vi "2_Analog_Meter_Reader(Evaluation).vi"() -> ()   [LabVIEW 2020]
uses:
  Controls/Regression_Report.ctl
  <vilib>/Ngene/Deep Learning Toolkit/Toolkit/NN_Network/Controls/NN_Save_Before_Destroy_Options.ctl
  <vilib>/Ngene/Deep Learning Toolkit/Toolkit/NN_Network/subVIs/NN_Predict/NN_Predict(In3D_Out1D).vi
  <vilib>/Ngene/Deep Learning Toolkit/Toolkit/Deep_Learning_Toolkit_by_Ngene.lvlib
panel:
  in  "Image Folder(Test)":path=path "D:/working/Analog_Meter/Test/Images"
  in  "Labels (Test)":path=path "D:/working/Analog_Meter/Test/Labels.csv"
  in  "NN Device":enum16{"CPU", "GPU"}(ring)=enum."GPU"
  in  "Image Folder(Train)":path=path "D:/working/Analog_Meter/Train/Images"
  in  "Labels (Train)":path=path "D:/working/Analog_Meter/Train/Labels.csv"
  out "Metrics (Test)":T1={"Graphs"=[{"Best Linear Fit"=[0.0, 0.7035179734230042, 1.407034993171692, 2.110553026199341, 2.814069986343384, 3.517587900161743, 4.221106052398682, 4.924623012542725, 5.628140926361084, 6.331657886505127, 7.035175800323486, 7.7386932373046875, 8.442211151123047, 9.145729064941406, 9.84924602508545, 10.552763938903809, 11.256280899047852, 11.959798812866211, 12.66331672668457, 13.366833686828613, 14.070351600646973, 14.773868560791016, 15.477387428283691, 16.180904388427734, 16.884422302246094, 17.587940216064453, 18.29145622253418, 18.99497413635254, 19.6984920501709, 20.402009963989258, 21.105527877807617, 21.809045791625977, 22.512563705444336, 23.216079711914062, 23.919597625732422, 24.62311553955078, 25.32663345336914, 26.0301513671875, 26.733667373657227, 27.437185287475586, 28.140703201293945, 28.844221115112305, 29.547739028930664, 30.251256942749023, 30.954774856567383, 31.65829086303711, 32.36180877685547, 33.06532669067383, 33.76884460449219, 34.47236251831055, 35.175880432128906, 35.879398345947266, 36.582916259765625, 37.28643035888672, 37.98994827270508, 38.69346618652344, 39.3969841003418, 40.100502014160156, 40.804019927978516, 41.507537841796875, 42.211055755615234, 42.914573669433594, 43.61809158325195, 44.32160949707031, 45.02512741088867, 45.728641510009766, 46.432159423828125, 47.135677337646484, 47.839195251464844, 48.5427131652832, 49.24623107910156, 49.94974899291992, 50.65326690673828, 51.35678482055664, 52.060302734375, 52.76382064819336, 53.46733856201172, 54.17085266113281, 54.87437057495117, 55.57788848876953, 56.28140640258789, 56.98492431640625, 57.68844223022461, 58.39196014404297, 59.09547805786133, 59.79899597167969, 60.50251388549805, 61.206031799316406, 61.909549713134766, 62.61306381225586, 63.31658172607422, 64.02010345458984, 64.72361755371094, 65.42713928222656, 66.13065338134766, 66.83416748046875, 67.53768920898438, 68.24120330810547, 68.9447250366211, 69.64823913574219, 70.35176086425781, 71.0552749633789, 71.75879669189453, 72.46231079101562, 73.16583251953125, 73.86934661865234, 74.57286071777344, 75.27638244628906, 75.97989654541016, 76.68341827392578, 77.38693237304688, 78.0904541015625, 78.7939682006836, 79.49748992919922, 80.20100402832031, 80.90452575683594, 81.60803985595703, 82.31156158447266, 83.01507568359375, 83.71858978271484, 84.42211151123047, 85.12562561035156, 85.82914733886719, 86.53266143798828, 87.2361831665039, 87.939697265625, 88.64321899414062, 89.34673309326172, 90.05024719238281, 90.75376892089844, 91.45728302001953, 92.16080474853516, 92.86431884765625, 93.56784057617188, 94.27135467529297, 94.9748764038086, 95.67839050292969, 96.38191223144531, 97.0854263305664, 97.78894805908203, 98.49246215820312, 99.19597625732422, 99.89949798583984, 100.60301208496094, 101.30653381347656, 102.01004791259766, 102.71356964111328, 103.41708374023438, 104.12060546875, 104.8241195678711, 105.52764129638672, 106.23115539550781, 106.9346694946289, 107.63819122314453, 108.34170532226562, 109.04522705078125, 109.74874114990234, 110.45226287841797, 111.15577697753906, 111.85929870605469, 112.56281280517578, 113.2663345336914, 113.9698486328125, 114.67337036132812, 115.37688446044922, 116.08039855957031, 116.78392028808594, 117.48743438720703, 118.19095611572266, 118.89447021484375, 119.59799194335938, 120.30150604248047, 121.0050277709961, 121.70854187011719, 122.41206359863281, 123.1155776977539, 123.819091796875, 124.52261352539062, 125.22612762451172, 125.92964935302734, 126.63316345214844, 127.33668518066406, 128.0402069091797, 128.74371337890625, 129.44723510742188, 130.1507568359375, 130.85427856445312, 131.5577850341797, 132.2613067626953, 132.96482849121094, 133.6683349609375, 134.37185668945312, 135.07537841796875, 135.77890014648438, 136.48240661621094, 137.18592834472656, 137.8894500732422, 138.5929718017578, 139.29647827148438, 140.0], "Array 3"=[2.1188226, 0.6589031, 1.929399, 2.432055, 2.4883072, 4.273648, 4.5083437, 5.706398, 5.9845705, 6.8059487, 7.432598, 7.994937, 8.78134, 9.417916, 10.277919, 10.736919, 11.286387, 11.683645, 13.034748, 13.586398, 14.125502, 15.080678, 15.584784, 16.422787, 17.089712, 17.690838, 17.784813, 18.926296, 19.709845, 20.683924, 21.649845, 22.522131, 22.717022, 22.988167, 23.577866, 24.204796, 25.393421, 25.715101, 26.404657, 27.686317, 28.289326, 28.841589, 29.523317, 30.209864, 31.038189, 31.62104, 32.218918, 32.86568, 33.492226, 33.975018, 35.333164, 36.030624, 36.599304, 37.123245, 37.91281, 38.50647, 39.085773, 39.85792, 40.96582, 41.15784, 41.639145, 42.434624, 43.35258, 44.505047, 45.25479, 46.004475, 46.779327, 47.277832, 47.861965, 48.508224, 48.970665, 49.554684, 50.45885, 51.149567, 52.214775, 52.91149, 53.535484, 54.2692, 55.005424, 55.659153, 56.401833, 56.88768, 57.88916, 58.370445, 59.22025, 59.84033, 60.424416, 61.191326, 61.82804, 62.630703, 63.13528, 64.011055, 64.73326, 65.51304, 66.41066, 67.34145, 67.8642, 68.267624, 69.247025, 69.374054, 70.29242, 71.4705, 72.27113, 72.63514, 73.22334, 74.1789, 74.79071, 75.46382, 76.0464, 76.79272, 77.32794, 77.795815, 78.34952, 79.27538, 80.03403, 80.65024, 81.92115, 82.61013, 83.241745, 83.793884, 84.675995, 85.672966, 86.3496, 86.88513, 87.43958, 88.04053, 89.190544, 90.360306, 90.99581, 91.4058, 91.692024, 91.96738, 92.47056, 93.27053, 93.939445, 94.78347, 95.663124, 96.47722, 97.483086, 97.98357, 98.58458, 98.99364, 99.654144, 100.27281, 100.90177, 102.2082, 102.532715, 102.93065, 103.456696, 103.85712, 105.56393, 106.15371, 106.93291, 107.80965, 108.29768, 109.04674, 109.87249, 110.62822, 111.24165, 111.70335, 112.376274, 113.187935, 113.69866, 114.51671, 115.66236, 116.61186, 117.31742, 117.53223, 117.78139, 118.74351, 119.38972, 120.17767, 120.90461, 121.91789, 122.35366, 123.190186, 123.76372, 124.78726, 125.52582, 125.96348, 126.331276, 127.12903, 128.17912, 128.88647, 129.19507, 129.93562, 130.9175, 130.79819, 131.62247, 133.0474, 133.42068, 134.0507, 134.65678, 135.86343, 136.04608, 137.67035, 137.70903, 138.1547, 138.02644, 138.06976]}, {"Best Linear Fit"=[1.920118723467626, 0.456393847942531, 1.7302014113306525, 2.234167616289601, 2.2905664843931697, 4.080560696728129, 4.315868365985859, 5.517045525403783, 5.795943102197606, 6.6194623359499145, 7.247745138585171, 7.811549758789713, 8.600002296688189, 9.238238248527674, 10.10048244691285, 10.560679464305368, 11.111579746966294, 11.509873043163736, 12.864497653827364, 13.417585630938483, 13.958094364960997, 14.915760479013052, 15.42118004741793, 16.261367543190772, 16.93003137985913, 17.532723990004126, 17.626944012347625, 18.771402707127898, 19.556993457662116, 20.533611622281153, 21.502050792876176, 22.3766103341453, 22.572009312489858, 22.843860945051397, 23.43509684413774, 24.063661235940646, 25.25538483983888, 25.577903399374055, 26.269256916681858, 27.55425776900406, 28.158837839308443, 28.712540627403598, 29.396045982103374, 30.084381857940546, 30.91486624039147, 31.499236909516107, 32.09867283815002, 32.74712153667766, 33.3752996397752, 33.859349984724076, 35.22103679434274, 35.92031496707152, 36.49047709619185, 37.01578383980195, 37.80740796095711, 38.40261383703523, 38.983427590357984, 39.75758840231808, 40.8683749608405, 41.06089589709805, 41.54345463219452, 42.34100694635282, 43.26135699777041, 44.416826832973946, 45.16852553041309, 45.920163033601895, 46.69703551578084, 47.196839555555485, 47.78249530393758, 48.43043914989979, 48.89408503699591, 49.47962604615859, 50.386150021636595, 51.07866622970115, 52.14665123474088, 52.84518360254346, 53.470803021048035, 54.2064305784877, 54.94457474947321, 55.60000724182262, 56.34462270478318, 56.83173658689045, 57.835827145278245, 58.318366757171475, 59.1703857787864, 59.79208111598695, 60.37769096868128, 61.14660054903278, 61.784975144095725, 62.58972925659268, 63.095622124277654, 63.973679299418635, 64.69776791602573, 65.4795780092802, 66.37953890140763, 67.31275886860301, 67.8368646750499, 68.241343371334, 69.22329690965587, 69.35065744320725, 70.2714167311741, 71.45256520368285, 72.25528843199616, 72.62024329183221, 73.20997993178486, 74.1680294660618, 74.78143298233924, 75.45629847381701, 76.04039759345571, 76.78865793895304, 77.32527796959752, 77.79437014497523, 78.3495167349147, 79.27779526639392, 80.03841685046297, 80.65623400204727, 81.93045892934602, 82.6212349259161, 83.25449597643376, 83.80807446370787, 84.69248436696384, 85.69205420010665, 86.37045365954243, 86.90737966143868, 87.463275880945, 88.06578682065926, 89.2188012365673, 90.39161199246519, 91.02877417644297, 91.43983125464024, 91.72680169168012, 92.00287190287551, 92.5073649520836, 93.3094226929243, 93.98008107969017, 94.82630577072459, 95.70825260540376, 96.52446916592034, 97.5329580610524, 98.03474326468229, 98.63732304792819, 99.04744691380755, 99.70967579258702, 100.32995601274811, 100.96055511337532, 102.2703874450994, 102.59574962495576, 102.9947208387079, 103.52213878395526, 103.92360366340938, 105.63486262818111, 106.22618266936169, 107.00741141723779, 107.88643622646251, 108.37574545230126, 109.12675188978328, 109.95465655211767, 110.71235611073226, 111.32738892392541, 111.79028518145468, 112.46496709018139, 113.27874352996507, 113.7908017183733, 114.61098060660038, 115.75961963360803, 116.71159563853723, 117.41899352335999, 117.6343590382032, 117.88416926671499, 118.84879718290509, 119.49669130853889, 120.28670143134093, 121.01553260235053, 122.03145659890073, 122.46836059859172, 123.30706604611376, 123.88209311813732, 124.90830539802846, 125.6487864244494, 126.08758744590138, 126.45634399854075, 127.25617579852478, 128.30900757732033, 129.01820304324727, 129.32760117304227, 130.07008631116233, 131.0545182166236, 130.9348987557421, 131.76132710678667, 133.18996807557502, 133.56423211074633, 134.19589446147347, 134.80355336749884, 136.01334839845504, 136.19647219264246, 137.8249735830903, 137.8637554392528, 138.31058055678258, 138.1819961382241, 138.22542875741357], "Array 3"=[2.1188226, 0.6589031, 1.929399, 2.432055, 2.4883072, 4.273648, 4.5083437, 5.706398, 5.9845705, 6.8059487, 7.432598, 7.994937, 8.78134, 9.417916, 10.277919, 10.736919, 11.286387, 11.683645, 13.034748, 13.586398, 14.125502, 15.080678, 15.584784, 16.422787, 17.089712, 17.690838, 17.784813, 18.926296, 19.709845, 20.683924, 21.649845, 22.522131, 22.717022, 22.988167, 23.577866, 24.204796, 25.393421, 25.715101, 26.404657, 27.686317, 28.289326, 28.841589, 29.523317, 30.209864, 31.038189, 31.62104, 32.218918, 32.86568, 33.492226, 33.975018, 35.333164, 36.030624, 36.599304, 37.123245, 37.91281, 38.50647, 39.085773, 39.85792, 40.96582, 41.15784, 41.639145, 42.434624, 43.35258, 44.505047, 45.25479, 46.004475, 46.779327, 47.277832, 47.861965, 48.508224, 48.970665, 49.554684, 50.45885, 51.149567, 52.214775, 52.91149, 53.535484, 54.2692, 55.005424, 55.659153, 56.401833, 56.88768, 57.88916, 58.370445, 59.22025, 59.84033, 60.424416, 61.191326, 61.82804, 62.630703, 63.13528, 64.011055, 64.73326, 65.51304, 66.41066, 67.34145, 67.8642, 68.267624, 69.247025, 69.374054, 70.29242, 71.4705, 72.27113, 72.63514, 73.22334, 74.1789, 74.79071, 75.46382, 76.0464, 76.79272, 77.32794, 77.795815, 78.34952, 79.27538, 80.03403, 80.65024, 81.92115, 82.61013, 83.241745, 83.793884, 84.675995, 85.672966, 86.3496, 86.88513, 87.43958, 88.04053, 89.190544, 90.360306, 90.99581, 91.4058, 91.692024, 91.96738, 92.47056, 93.27053, 93.939445, 94.78347, 95.663124, 96.47722, 97.483086, 97.98357, 98.58458, 98.99364, 99.654144, 100.27281, 100.90177, 102.2082, 102.532715, 102.93065, 103.456696, 103.85712, 105.56393, 106.15371, 106.93291, 107.80965, 108.29768, 109.04674, 109.87249, 110.62822, 111.24165, 111.70335, 112.376274, 113.187935, 113.69866, 114.51671, 115.66236, 116.61186, 117.31742, 117.53223, 117.78139, 118.74351, 119.38972, 120.17767, 120.90461, 121.91789, 122.35366, 123.190186, 123.76372, 124.78726, 125.52582, 125.96348, 126.331276, 127.12903, 128.17912, 128.88647, 129.19507, 129.93562, 130.9175, 130.79819, 131.62247, 133.0474, 133.42068, 134.0507, 134.65678, 135.86343, 136.04608, 137.67035, 137.70903, 138.1547, 138.02644, 138.06976]}, {"Best Linear Fit"=[0.0, 140.0], "Array 3"=[0.0, 140.0]}], "y=k*x+b"="y = 0.997*x + 0.204", "R"=0.9999598, "R^2"=0.99991965, "MAE"=0.26860958, "MSE"=0.1448541} {"R" format="%#_7g"}
  out "Metrics (Train)":T1={"Graphs"=[{"Best Linear Fit"=array[1000 elements], "Array 3"=array[1000 elements]}, {"Best Linear Fit"=array[1000 elements], "Array 3"=array[1000 elements]}, {"Best Linear Fit"=[0.0, 140.0], "Array 3"=[0.0, 140.0]}], "y=k*x+b"="y = 0.998*x + 0.138", "R"=0.99996376, "R^2"=0.9999275, "MAE"=0.2552316, "MSE"=0.12359543} {"R" format="%#_7g"}
  in  "Network Configuration File Path":path=path "D:/Ngene/GitHub/deepltk_examples/3_Image_Processing/31_Image_Regression/working/Analog_Meter/Analog_Meter_net_cfg_24_01_29__18_13_27.cfg"
  in  "Weight File Path":path=path "D:/Ngene/GitHub/deepltk_examples/3_Image_Processing/31_Image_Regression/working/Analog_Meter/Analog_Meter_weights_24_01_29__18_13_27.bin"
  # "Overview: Performs evaluation of a trained model over Training and Tests Datasets\nInstructions:\n1. Provide paths to Train and Test datasets \n2. Provide model files (.cfg and .bin).\n2. Run the VI\n3. Drag and drop image on \"Input Image\"\n4. Observe calculated metrics on both train and test datasets."
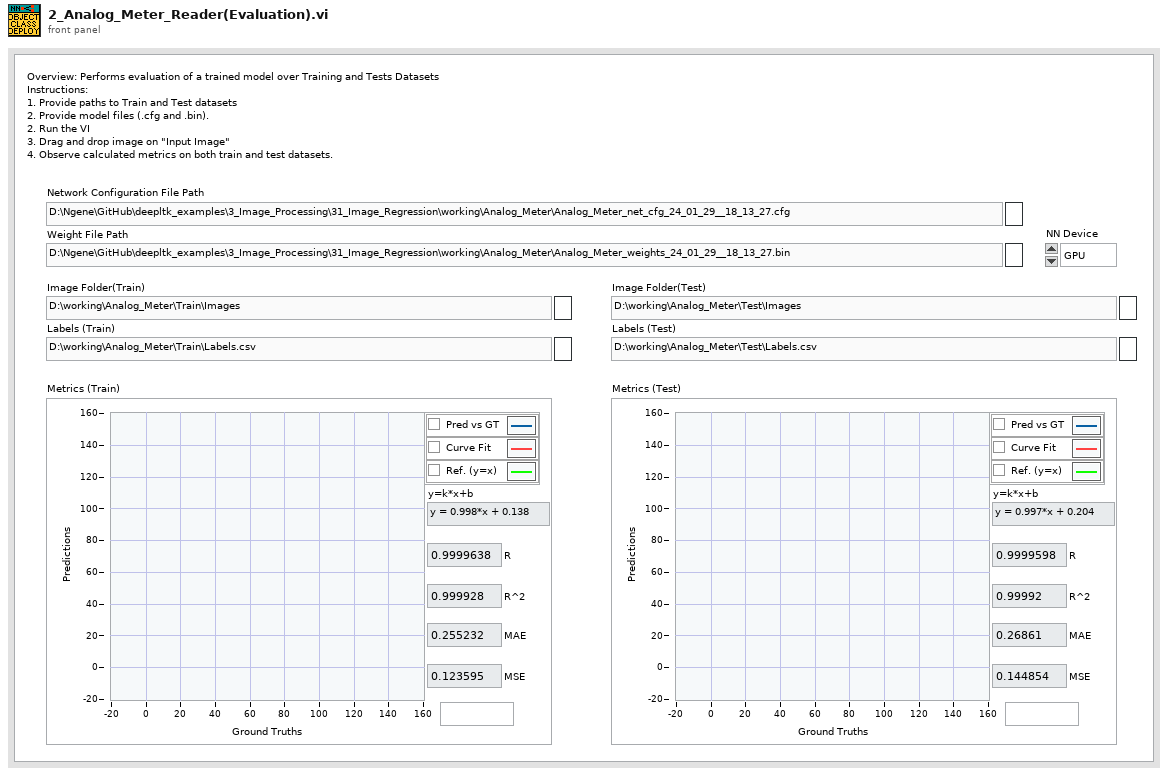
[diagram p1: front panel]
types:
  T1 = typedef "Regression_Report.ctl" = cluster{"Graphs":cluster{"Best Linear Fit":dbl[], "Array 3":sgl[]}[], "y=k*x+b":string, "R":sgl, "R^2":sgl, "MAE":sgl, "MSE":sgl}
  T2 = typedef "Deep_Learning_Toolkit_by_Ngene.lvlib/NN_Save_Before_Destroy_Options.ctl" = cluster{"CFG?":bool, "Weights?":bool, "Render?":bool}
  T3 = typedef "Deep_Learning_Toolkit_by_Ngene.lvlib/NN_Config_Params.ctl" = cluster{"Name":string, "mBatch":i32, "NN_Train_Params":T4, "LR_Decay_Policy":T7, "Labels":string[], "Loss":T9, "Max_WS_Size(B)":i64, "DryRun?":bool}
  T4 = typedef "Deep_Learning_Toolkit_by_Ngene.lvlib/NN_Train_Params.ctl" = cluster{"Optimizer":T5, "Beta_1":sgl, "Beta_2":sgl, "Weight Decay(L1)":sgl, "Weight Decay(L2)":sgl, "Data_Sampling":T6}
  T5 = typedef "Deep_Learning_Toolkit_by_Ngene.lvlib/NN_Train_Optimizer.ctl" = enum16{"SGD", "Adam", "Adagrad", "Adadelta", "RMSProp", "Nesterov"}
  T6 = typedef "Deep_Learning_Toolkit_by_Ngene.lvlib/NN_Train_Data_Sampling.ctl" = enum16{"Random", "Sequential"}
  T7 = typedef "Deep_Learning_Toolkit_by_Ngene.lvlib/NN_LR_Policy_Cfg.ctl" = cluster{"Policy_Type":T8, "LR0":dbl, "k":sgl, "WarmUp_Policy":enum16{"Step", "Ramp"}, "WarmUp_Iter":i32, "WarmUp_Ratio":sgl}
  T8 = typedef "Deep_Learning_Toolkit_by_Ngene.lvlib/NN_LR_Policy_Type.ctl" = enum16{"Manual", "Step", "Exp", "1/t"}
  T9 = typedef "Deep_Learning_Toolkit_by_Ngene.lvlib/NN_Loss_Config_Params.ctl" = cluster{"Loss_Type":T10, "Loss_Conf_Params":variant}
  T10 = typedef "Deep_Learning_Toolkit_by_Ngene.lvlib/NN_Loss_Type.ctl" = enum16{"None", "MSE", "CrossEntropy", "YOLO_v2", "YOLO_v4"}
  T11 = typedef "Deep_Learning_Toolkit_by_Ngene.lvlib/NN_Layer_Config_Params.ctl" = cluster{"Layer_Type":T12, "Layer_Conf_Params":variant, "Input Layers":string[]}
  T12 = typedef "Deep_Learning_Toolkit_by_Ngene.lvlib/NN_Layer_Type.ctl" = enum16{"Input1D", "Input3D", "Conv1D", "Conv2D", "Conv2D_Adv", "MaxPool", "AvgPool", "UpSample", "DropOut3D", "ShortCut", "Concat", "SoftMax3D", "FC", "DropOut", "Softmax", "Flatten", "YOLO_v2", "YOLO_v4", "Activation", "BatchNormalization", "LayerNormalization", "Scale", "Unsupported"}
  T13 = typedef "Deep_Learning_Toolkit_by_Ngene.lvlib/NN.ctl" = cluster{"Name":string, "No of Layers":i32, "mBatch":i32, "Layers":T14[], "Dimty":T15, "Dims_In":T16, "Dims_Out":T16, "Working_Dir":path, "Train?":bool, "Train_Params":T4, "LR_Update_Policy":T7, "Session Data":T17, "Ground_truth":T18, "NNg_hdls":T19, "NN_Device":T20, "GPU Id":i32, "Labels":string[], "Loss_Type":T10, "Loss_Cfg_Prms":variant, "NNG_WS":T21, "DryRun?":bool}
  T14 = typedef "Deep_Learning_Toolkit_by_Ngene.lvlib/NN_Layer_ref.ctl" = refnum<file>
  T15 = typedef "Deep_Learning_Toolkit_by_Ngene.lvlib/NN_In_Out_Dim-ty.ctl" = enum8{"In1D_Out1D", "In3D_Out1D", "In3D_Out3D", "In3D_OutBBox"}
  T16 = typedef "Deep_Learning_Toolkit_by_Ngene.lvlib/NN_Dims(C,H,W).ctl" = cluster{"C":i32, "H":i32, "W":i32}
  T17 = typedef "Deep_Learning_Toolkit_by_Ngene.lvlib/NN_Train_Session_Data.ctl" = cluster{"Epochs":sgl, "Tot_Iter":i32, "LR":sgl, "LR_iter":i32}
  T18 = typedef "Deep_Learning_Toolkit_by_Ngene.lvlib/NN_Ground_truth.ctl" = cluster{"Y":variant}
  T19 = typedef "Deep_Learning_Toolkit_by_Ngene.lvlib/nng_cuda_handles.ctl" = cluster{"cudnn":u64, "cublas":u64, "stream":u64, "curand":u64}
  T20 = typedef "Deep_Learning_Toolkit_by_Ngene.lvlib/NN_Device.ctl" = enum16{"CPU", "GPU"}
  T21 = typedef "Deep_Learning_Toolkit_by_Ngene.lvlib/NNG_WS.ctl" = cluster{"NNG_WS_Mem":T22, "Max_WS_Size":i64}
  T22 = typedef "Deep_Learning_Toolkit_by_Ngene.lvlib/NNg_WS_Mem_DVR.ctl" = refnum<data-value>
  T23 = typedef "Deep_Learning_Toolkit_by_Ngene.lvlib/NN_DataSets_All(In3D_Out1D).ctl" = cluster{"Train":T24, "Validation":T24, "Test":T24}
  T24 = typedef "Deep_Learning_Toolkit_by_Ngene.lvlib/NN_DataSet(In3D_Out1D).ctl" = cluster{"Inputs Ref.":variant, "Outputs Ref.":T25, "Dataset_Size":i32, "Dims_In":T16, "Dims_Out":i32, "Labels":string[], "File Paths":path[], "Custom_Data":variant}
  T25 = typedef "Deep_Learning_Toolkit_by_Ngene.lvlib/NN_Data_ref(2D_SGL).ctl" = refnum<data-value>
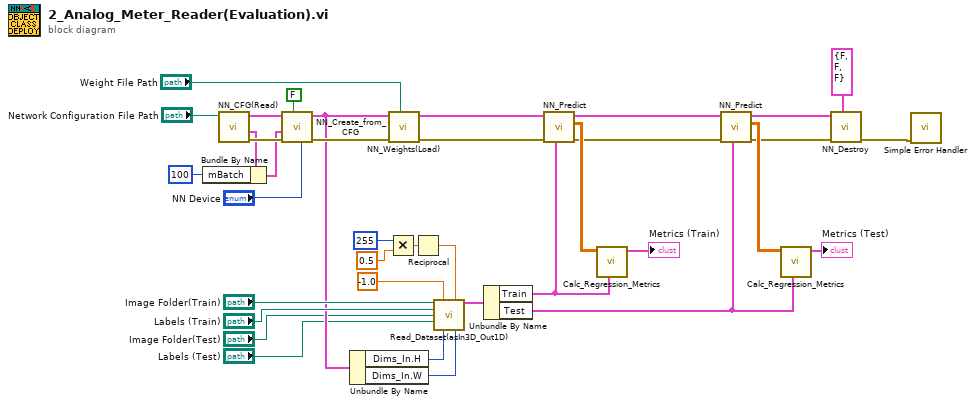
[diagram p0: block diagram]
diagram:
  n1 = call <vilib>:"NN_CFG(Read).vi"("CFG file path"="Network Configuration File Path") -> ("error out"=w37:errorcluster, "Net_Cfg"=w31:T3, "Layer_Cfg"=w30:T11[])  [unwired: 8 in]
  n2 = Bundle By Name(cluster=w31, "mBatch"=100) -> (w28:T3)
  n3 = call <vilib>:"NN_Create_from_CFG.vi"("NN_Device"="NN Device", "Train? (false)"=FALSE, "error in (no error)"=w37, "Net_Cfg"=w28, "Layer_Cfg"=w30) -> ("error out"=w33:errorcluster, "NN out"=w9:T13)  [unwired: 5 in]
  n4 = Unbundle By Name(w9) -> ("Dims_In.H"=w8:i32, "Dims_In.W"=w7:i32)
  n5 = Multiply(x=u16 255 ("Shift"), y=sgl 0.5 ("Scale")) -> (x*y=w23:sgl)
  n6 = call <vilib>:"NN_Weights(Load).vi"("Weight File Path"="Weight File Path", "error in (no error)"=w33, "NN in"=w9) -> ("error out"=w19:errorcluster, "NN out"=w29:T13)  [unwired: 7 in]
  n7 = Reciprocal(x=w23) -> (1/x=w22:sgl)
  n8 = call "Read_Dataset(asIn3D_Out1D).vi"("Image Folder Path(Train)"="Image Folder(Train)", "Norm. Shift"=sgl -1.0 ("Scale"), "Norm. Scale"=w22, "Label File Path(Train)"="Labels (Train)", "Image Folder Path(Test)"="Image Folder(Test)", "Label File Path(Test)"="Labels (Test)", "Img Heigth"=w8, "Img Width"=w7) -> ("Datasets"=w20:T23)  [unwired: 6 in, 1 out]
  n9 = Unbundle By Name(w20) -> ("Train"=w6:T24, "Test"=w5:T24)
  n10 = call-poly <vilib>:"NN_Predict.vi"("Dataset"=w6, "error in (no error)"=w19, "NN in"=w29) -> ("error out"=w14:errorcluster, "Predictions"=w21:sgl[][], "NN out"=w15:T13)  [unwired: 6 in]
  n11 = call "Calc_Regression_Metrics.vi"("Dataset"=w6, "Predictions"=w21) -> ("Metrics"=→"Metrics (Train)":T1)  [unwired: 9 in]
  n12 = call-poly <vilib>:"NN_Predict.vi"("Dataset"=w5, "error in (no error)"=w14, "NN in"=w15) -> ("error out"=w17:errorcluster, "Predictions"=w18:sgl[][], "NN out"=w16:T13)  [unwired: 6 in]
  n13 = call "Calc_Regression_Metrics.vi"("Dataset"=w5, "Predictions"=w18) -> ("Metrics"=→"Metrics (Test)":T1)  [unwired: 9 in]
  n14 = call <vilib>:"NN_Destroy.vi"("Save (T, T, T)"=T2 {"CFG?"=FALSE, "Weights?"=FALSE, "Render?"=FALSE} ("Save_Config"), "error in (no error)"=w17, "NN in"=w16) -> ("error out"=w35:errorcluster)  [unwired: 7 in, 1 out]
  n15 = call <vilib>:"Simple Error Handler.vi"("error in (no error)"=w35) -> ()  [unwired: 4 in, 5 out]
